vi "Client Send Request.vi"(6 "Reply?":bool, 8 "error in (no error)":errorcluster caption="错误输入（无错误）", 9 "Data输入":variant, 10 "命令":string) -> (0 "error out":errorcluster caption="错误输出", 1 "有效?":bool, 2 "Data输出":variant)   [LabVIEW 2020, in "TCP Communication.lvlib"]
uses:
  TCP Communication.lvlib
  Reply.ctl
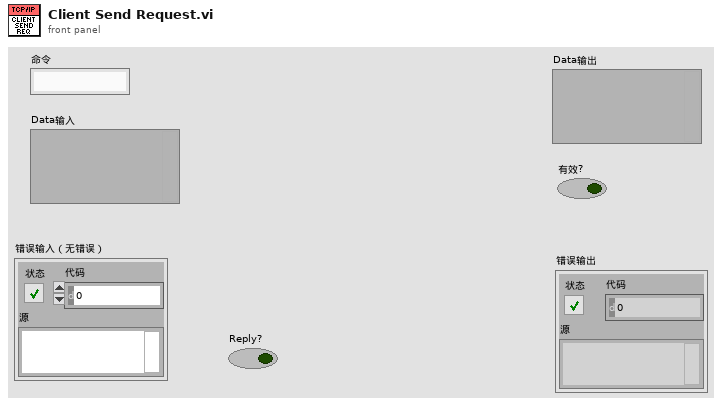
[diagram p1: front panel]
types:
  T1 = cluster{"Send Queue":refnum<queue>, "Received Reply Queue":refnum<queue>}
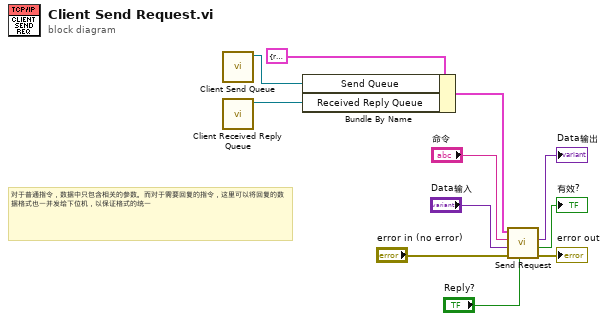
[diagram p0: block diagram]
diagram:
  # "对于普通指令，数据中只包含相关的参数。而对于需要回复的指令，这里可以将回复的数据格式也一并发给下位机，以保证格式的统一"
  n1 = call "Client Send Queue.vi"() -> ("发送队列"=w6:refnum<queue>)  [unwired: 10 in, 1 out]
  n2 = call "Client Received Reply Queue.vi"() -> ("queue out"=w5:refnum<queue>)  [unwired: 10 in, 1 out]
  n3 = Bundle By Name(cluster=T1 {"Send Queue"=refnum, "Received Reply Queue"=refnum} ("Queues"), "Send Queue"=w6, "Received Reply Queue"=w5) -> (w7:T1)
  n4 = call "Send Request.vi"("Reply?"="Reply?", "error in (no error)"="error in (no error)", "Data输入"="Data输入", "命令"="命令", "Queues"=w7) -> ("error out"=→"error out":errorcluster, "有效?"=→"有效?":bool, "Data输出"=→"Data输出":variant)  [unwired: 4 in]
